vi "Update Scan Table.vi"(7 "Scan Table Ref":refnum<vi>, 8 "error in (no error)":errorcluster, 11 "Scanned Addresses Ref":refnum<vi>) -> (0 "error out":errorcluster)   [LabVIEW 2025, in "I2C Bus Monitor UI.lvlib"]
uses:
  I2C Bus Monitor UI.lvlib
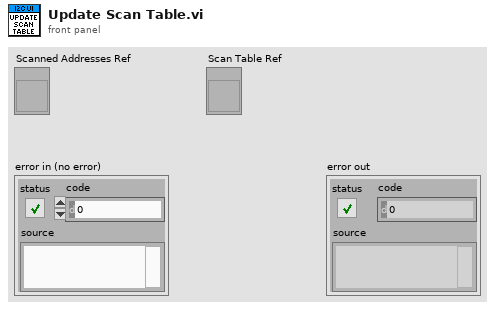
[diagram p1: front panel]
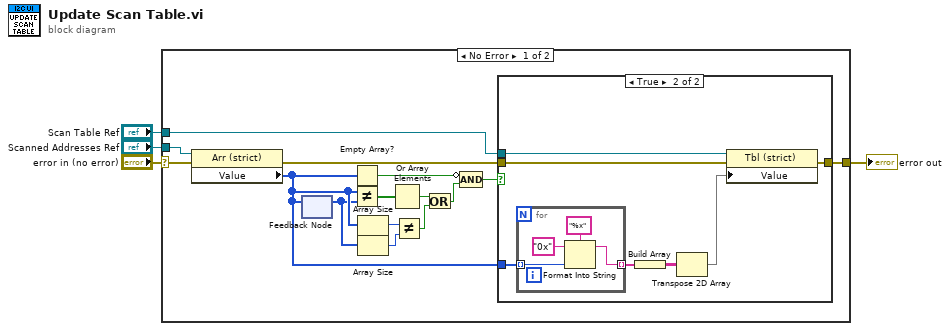
[diagram p0: block diagram]
diagram:
  n1 = case shown="No Error" "error in (no error)" {
    selector: "error in (no error)" -> [w19 w32]
    tunnel: [w18 w32] -> w3
    tunnel: "Scanned Addresses Ref" -> [w16 _]
    tunnel: "Scan Table Ref" -> [w15 _]
    frame No Error {
      n2 = property class="Arr (strict)"(reference=w16, error in=w19) -> (error out=w17:errorcluster, "Value"=w9:i32[])  [unwired: 1 out]
      n3 = feedback #1() -> (w8:i32[])  [unwired: 1 in]
      n4 = feedback-in #1(w9) -> ()
      n5 = Empty Array?(array=w9) -> (empty?=w13:bool)
      n6 = Not Equal?(x=w9, y=w8) -> (x != y?=w14:bool[])
      n7 = Array Size(array=w9) -> (size(s)=w7:i32)
      n8 = Array Size(array=w8) -> (size(s)=w6:i32)
      n9 = Or Array Elements(Boolean array=w14) -> (logical OR=w11:bool)
      n10 = Not Equal?(x=w7, y=w6) -> (x != y?=w5:bool)
      n11 = Or(x=w11, y=w5) -> (x .or. y?=w10:bool)
      n12 = Compound Arithmetic op=AND(invert w13, w10) -> (w12:bool)
      n13 = case shown="True" w12 {
        tunnel: [w20 w27] -> w18
        tunnel: w17 -> [w20 w26]
        tunnel: w9 -> [_ w25]
        tunnel: w15 -> [_ w24]
        frame False {
        }
        frame True {
          n14 = for {
            tunnel: w25 -> [w29] mode=indexing
            tunnel: [w28] -> w22 mode=indexing
            n15 = Format Into String(format string="%x", initial string="0x", w29) -> (resulting string=w28:string)  [unwired: 1 in, 1 out]
          }
          n16 = Build Array(w22) -> (w23:string[][])
          n17 = Transpose 2D Array(2D array=w23) -> (transposed array=w21:string[][])
          n18 = property class="Tbl (strict)"(reference=w24, error in=w26, "Value"=w21) -> (error out=w27:errorcluster)  [unwired: 1 out]
        }
      }
    }
    frame Error {
    }
  }
  "error out" <- w3
